vi "nof.vi"() -> ()   [LabVIEW 2023]
panel:
  out "data":cluster{timestamp[], dbl[]}(graph)
  in  "reference value (0)":dbl format="%.5f"
  in  "post-notch gain\n(auto select)":u16(ring) items=["automatic selection", "0dB", "20dB", "40dB", "60dB"]
  in  "notch tune\n(false:automatic)":bool
  in  "post-notch detector response\n(fast rms)":u16(ring) items=["no change", "fast rms", "slow rms", "fast avg", "slow avg"]
  in  "low pass filters\n(30kHz)":u16(ring)=1 items=["off(750kHz) ", "low pass 30kHz", "low pass 80 kHz"]
  in  "HP/BP filter\n(off)":u16(ring) items=["off ", "left HP/BP filter", "right HP/BP filter"]
  in  "frequency increment\n(1000Hz)":dbl=1000.0 format="%.5f"
  in  "amplitude increment\n(.1V)":dbl=0.1 format="%.5f"
  in  "source frequency\n(1000Hz)":dbl=1000.0 min=10.0 max=100000.0 format="%.5f"
  in  "output impedance\n(f:60 ohms)":bool
  in  "source amplitude\n(.6mV)":dbl=0.0006 min=0.0006 max=6.0 format="%.5f"
  in  "set reference value\n(no:f)":bool
  in  "measurement mode\n(LIN:f)":bool
  in  "detector selection\n(no change)":u16(ring) items=["no change", "rms", "average", "quasi-peak"]
  out "error out":errorcluster
  in  "measurements\n(AC level)":u16(ring) items=["AC level", "DC level", "Distortion", "Distortion level", "Signal-to-Noise", "SINAD"]
  out "value read":dbl format="%.7f"
  in  "stop":bool
  in  "error in (no error)":errorcluster
  in  "SINAD meter range\n(f:0 to 18)":bool
  in  "range selector\n(f:except DC)":bool
  in  "SPCL 2(spcial function 2)\ninput level range(DC only)\n(auto select)":u16(ring) items=["automatic select", "300V", "64V", "16V", "4V"]
  in  "SPCL 2(spcial function 1)\ninput level range(except DC)\n(auto select)":u16(ring) items=["automatic select", "300V", "189V", "119V", "75.4V", "47.6V", "30.0V", "18.9V", "11.9V", "7.54V", "4.76V", "3.00V", "1.89V", "1.19V", "0.754V", "0.476V", "0.300V", "0.189V", "0.119V", "0.0754V"]
  in  "VISA resource name":refnum<visa-resource-name>
  # "INPUT"
  # "OUTPUT"
  # "input range (DC only)"
  # "input range (except DC)"
  # "0 to 24 dB"
  # "0 to 18 dB"
  # "hold notch tuning"
  # "automatic notch tuning"
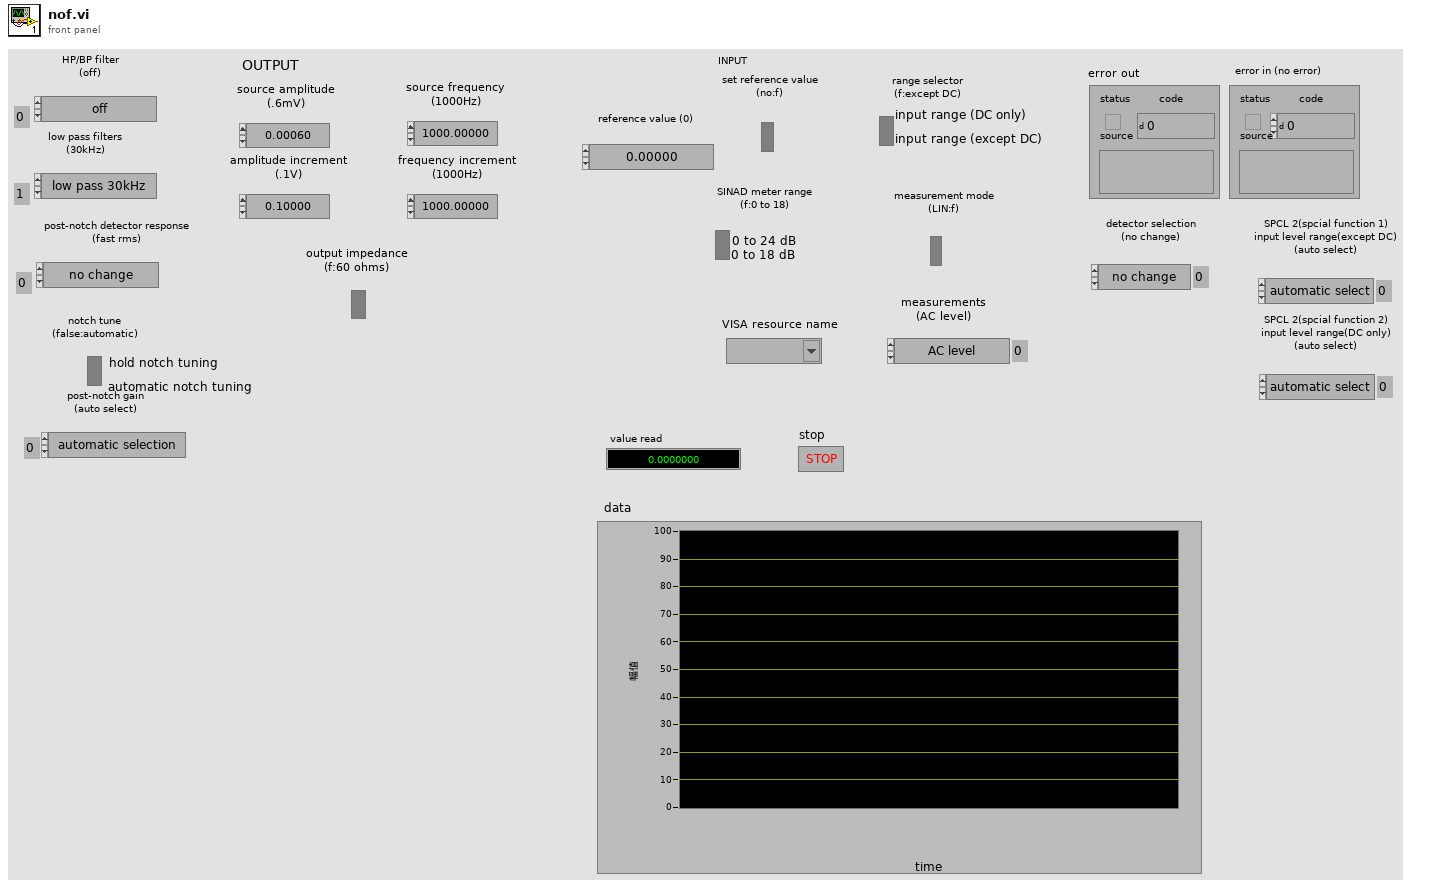
[diagram p1: front panel]
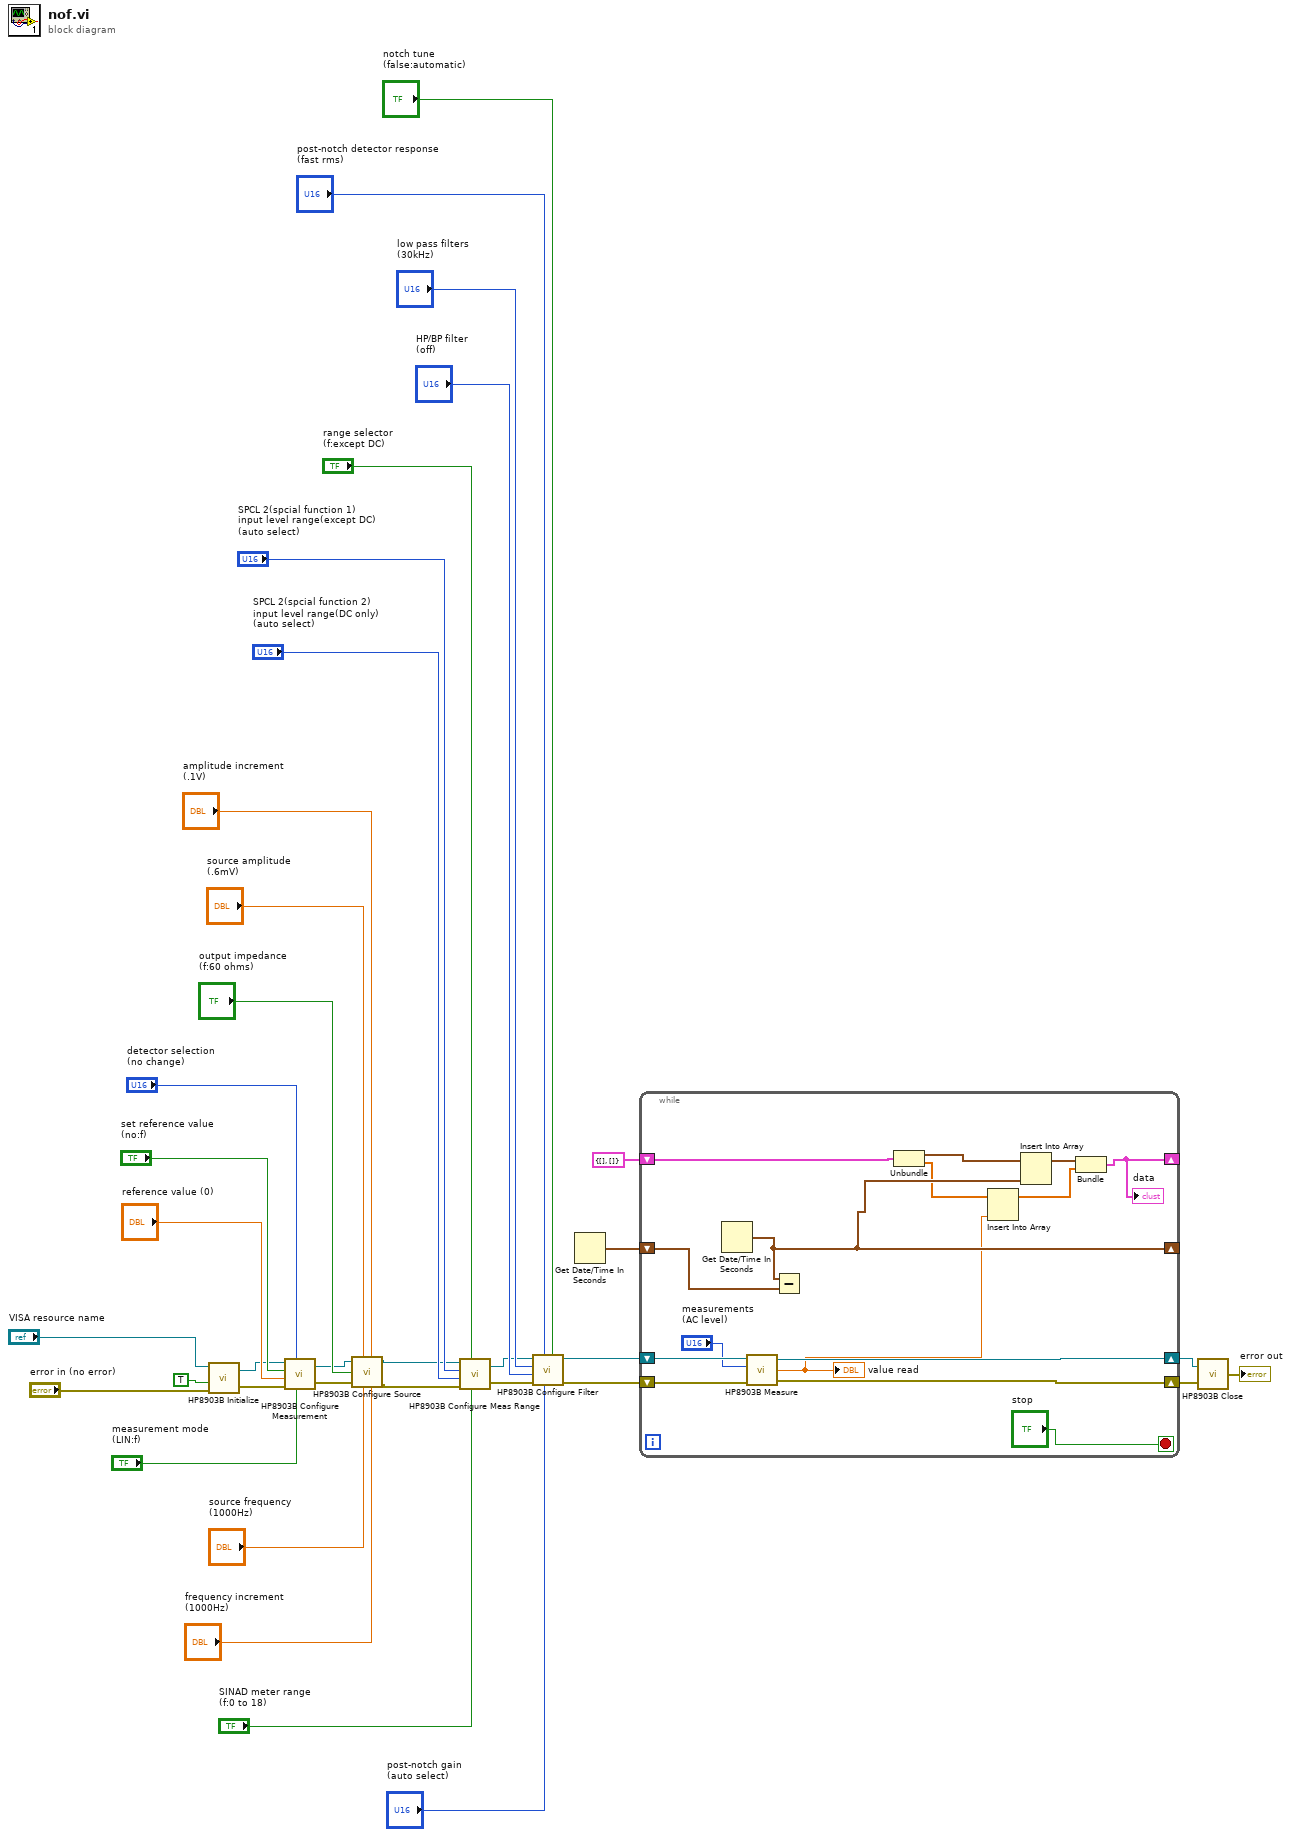
[diagram p0: block diagram]
diagram:
  n1 = call <instrlib>:"HP8903B Initialize.vi"("error in (no error)"="error in (no error)", "reset (no : F)"=TRUE, "VISA resource name"="VISA resource name") -> ("error out"=w9:errorcluster, "VISA session"=w10:refnum<visa-resource-name>)  [unwired: 1 in]
  n2 = call <instrlib>:"HP8903B Configure Measurement.vi"("measurement mode\n(LIN:f)"="measurement mode\n(LIN:f)", "detector selection\n(no change)"="detector selection\n(no change)", "error in (no error)"=w9, "reference value (0)"="reference value (0)", "set reference value\n(no:f)"="set reference value\n(no:f)", "VISA session"=w10) -> ("error out"=w7:errorcluster, "dup VISA session"=w8:refnum<visa-resource-name>)
  n3 = call <instrlib>:"HP8903B Configure Source.vi"("VISA session"=w8, "source amplitude\n(.6mV)"="source amplitude\n(.6mV)", "output impedence\n(f:60 ohms)"="output impedance\n(f:60 ohms)", "error in (no error)"=w7, "source frequency\n(1000Hz)"="source frequency\n(1000Hz)", "amplitude increment\n(.1V)"="amplitude increment\n(.1V)", "frequency increment\n(1000Hz)"="frequency increment\n(1000Hz)") -> ("dup VISA session"=w4:refnum<visa-resource-name>, "error out"=w3:errorcluster)  [unwired: 2 in]
  n4 = call <instrlib>:"HP8903B Configure Meas Range.vi"("SINAD meter range\n(f:0 to 18)"="SINAD meter range\n(f:0 to 18)", "range selector\n(f:except DC)"="range selector\n(f:except DC)", "error in (no error)"=w3, "input level range : DC only\n(auto select)"="SPCL 2(spcial function 2)\ninput level range(DC only)\n(auto select)", "input level range : except DC\n(auto select)"="SPCL 2(spcial function 1)\ninput level range(except DC)\n(auto select)", "VISA session"=w4) -> ("error out"=w5:errorcluster, "dup VISA session"=w6:refnum<visa-resource-name>)
  n5 = call <instrlib>:"HP8903B Configure Filter.vi"("notch tune\n(false:automatic)"="notch tune\n(false:automatic)", "post-notch gain\n(auto select)"="post-notch gain\n(auto select)", "post-notch detector response\n(fast rms)"="post-notch detector response\n(fast rms)", "error in (no error)"=w5, "HP/BP filter\n(off)"="HP/BP filter\n(off)", "low pass filters\n(30kHz)"="low pass filters\n(30kHz)", "VISA session"=w6) -> ("error out"=w11:errorcluster, "dup VISA session"=w12:refnum<visa-resource-name>)  [unwired: 2 in]
  n6 = Get Date/Time In Seconds() -> (seconds since 1Jan1904=w2:timestamp)
  n7 = while {
    shift-right: [w47] -> w14
    shift-left: w11 -> [w51]
    shift-right: [w48] -> w13
    shift-left: w12 -> [w50]
    shift-right: [w38] -> _
    shift-left: cluster{timestamp[], dbl[]} {[], []} ("输出簇") -> [w41]
    shift-right: [w42] -> _
    shift-left: w2 -> [w45]
    stop <- "stop" stop-if-true
    n8 = Get Date/Time In Seconds() -> (seconds since 1Jan1904=w42:timestamp)
    n9 = call <instrlib>:"HP8903B Measure.vi"("error in (no error)"=w51, "measurements\n(AC level)"="measurements\n(AC level)", "VISA session"=w50) -> ("error out"=w47:errorcluster, "value read"=w37:dbl, "dup VISA session"=w48:refnum<visa-resource-name>)  [unwired: 1 in]
    "value read" <- w37
    n10 = Subtract(x=w42, y=w45) -> ()  [unwired: 1 out]
    n11 = Unbundle(w41) -> (w40:timestamp[], w39:dbl[])
    n12 = Insert Into Array(array=w39, new element=w37) -> (w43:dbl[])  [unwired: 1 in]
    n13 = Insert Into Array(array=w40, new element=w42) -> (w44:timestamp[])  [unwired: 1 in]
    n14 = Bundle(w44, w43) -> (w38:cluster{timestamp[], dbl[]})  [unwired: 1 in]
    "data" <- w38
  }
  n15 = call <instrlib>:"HP8903B Close.vi"("error in (no error)"=w14, "VISA session"=w13) -> ("error out"=→"error out":errorcluster)
